vi "RT Driver VI.vi"(7 "Operation":T1, 11 "Device Reference in":T2 format="%.0x") -> (0 "Error Code":i32)   [LabVIEW 2020, in "AIM ARINC 429 Engine.lvlib" / "Custom Device.lvlib"]
uses:
  Custom Device.lvlib
  <vilib>/NI VeriStand/Custom Device API/Custom Device Item Ref.ctl
  <vilib>/NI VeriStand/Custom Device API/Hardware Interface Driver VI Operation.ctl
  Compiled.Settings.ctl
  Inline Execution Unit Compiled Information.ctl
  <vilib>/NI VeriStand/Custom Device API/Data Reference.ctl
  <vilib>/NI VeriStand/Custom Device API/Block Data Reference.ctl
  Asynchronous Execution Unit Compiled Information.ctl
  RTStateVariables.ctl
  <vilib>/NI/NIVS Inline Async API/_VS Inline Async API/VS Inline Async API/VS Inline Async API.lvclass
  Inline Execution Unit Runtime Information.ctl
  Interfaces/Execution Unit/Execution Unit.lvclass
  Asynchronous Execution Unit Runtime Information.ctl
  Interfaces/Shared Resources/Shared Resources.lvclass
  <vilib>/NI/NIVS Inline Async API/_VS Inline Async API/VS Inline Async API/VS Inline Async API.lvclass/VS Inline Async API.ctl
  <vilib>/NI/NIVS Inline Async API/_Data Access Engine/Data Access Engine/Data Access Engine.lvclass/Data Access Engine.ctl
  <vilib>/NI/NIVS Inline Async API/_Data Access Engine/Access Type Classes/Write/Write.lvclass/Write.ctl
  <vilib>/NI/NIVS Inline Async API/_Data Access Engine/Access Type Classes/ReadWrite/ReadWrite.lvclass/ReadWrite.ctl
  <vilib>/NI/NIVS Inline Async API/_Data Access Engine/Access Type Classes/Read/Read.lvclass/Read.ctl
  <vilib>/NI/NIVS Inline Async API/_Data Access Engine/Data Access Engine/Methods/Data.Engine.Read Data from HW.vi
  <vilib>/NI/NIVS Inline Async API/_VS Inline Async API/Error Handling Process/SubVIs/Error.GetError.vi
  <vilib>/NI/NIVS Inline Async API/_Data Access Engine/Data Access Engine/Methods/Data.Engine.Write Data to HW.vi
  <vilib>/NI/NIVS Inline Async API/_Data Access Engine/Access Type Classes/ReadWrite/ReadWrite.EngineData.vi
  <vilib>/NI/NIVS Inline Async API/_Data Access Engine/Access Type Classes/Write/Write.EngineData.vi
  <vilib>/NI/NIVS Inline Async API/_Data Access Engine/Access Type Classes/Read/Read.EngineData.vi
  <vilib>/NI VeriStand/Custom Device API/NI VeriStand - Get Channel Value by Data Reference.vi
  <vilib>/NI VeriStand/Custom Device API/NI VeriStand - Set Channel Value by Data Reference.vi
  <vilib>/NI VeriStand/Custom Device API/NI VeriStand - Get Channel Values by Block Data Reference.vi
  Scripting/AIM/Constants.vi
  <vilib>/NI VeriStand/Custom Device API/Get Item Property (Variant).vi
  <vilib>/NI VeriStand/Custom Device API/Global Data Refs.vi
  <vilib>/NI VeriStand/Custom Device API/Custom Device API.lvlib
  <vilib>/NI VeriStand/Custom Device Tools/Custom Device Utility Library/Custom Device Utility Library.lvlib
  Scripting/AIM/AIM ARINC 429 Scripting.lvlib
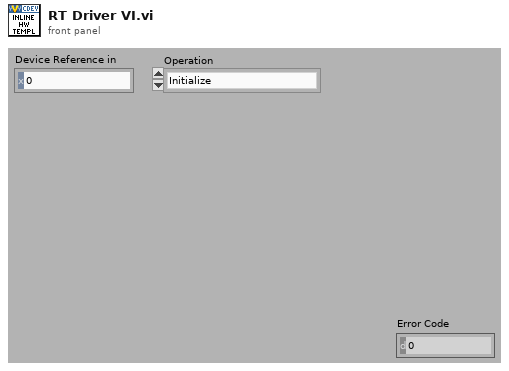
[diagram p1: front panel]
types:
  T1 = typedef "Custom Device API.lvlib/Hardware Interface Driver VI Operation.ctl" = enum16{"Initialize", "Start", "Read Data from HW", "Write Data to HW", "Close"}
  T2 = typedef "Custom Device API.lvlib/Custom Device Item Ref.ctl" = u64
  T3 = typedef "AIM ARINC 429 Engine.lvlib/Custom Device.lvlib/RTStateVariables.ctl" = cluster{"Async":refnum<class "VS Inline Async API.lvclass">, "Inline Execution Units":T4[], "Asynchronous Execution Units":cluster{"Grouped Asynchronous Execution Units":T7[]}[], "shared resources":refnum<class "Shared Resources.lvclass">}
  T4 = typedef "AIM ARINC 429 Engine.lvlib/Custom Device.lvlib/Inline Execution Unit Runtime Information.ctl" = cluster{"Execution Unit":refnum<class "Execution Unit.lvclass">, "Incoming Buffer":dbl[], "Outgoing Buffer":dbl[], "Incoming Data References":T5[], "Outgoing Data References":T6[]}
  T5 = typedef "Custom Device API.lvlib/Data Reference.ctl" = i32
  T6 = typedef "Custom Device API.lvlib/Block Data Reference.ctl" = cluster{"Data Reference":T5, "Offset":u64, "Length":u64}
  T7 = typedef "AIM ARINC 429 Engine.lvlib/Custom Device.lvlib/Asynchronous Execution Unit Runtime Information.ctl" = cluster{"Execution Unit":refnum<class "Execution Unit.lvclass">, "Incoming Channel Group Name":string, "Outgoing Channel Group Name":string, "ReadWrite Channel Group Name":string}
  T8 = typedef "AIM ARINC 429 Engine.lvlib/Custom Device.lvlib/Compiled.Settings.ctl" = cluster{"Name":string, "Inline Execution Unit Compiled Information":T9[], "Asynchronous Execution Unit Compiled Information":cluster{"Grouped Asynchronous Execution Unit Compiled Information":T10[]}[], "Flattened Shared Resources":string}
  T9 = typedef "AIM ARINC 429 Engine.lvlib/Custom Device.lvlib/Inline Execution Unit Compiled Information.ctl" = cluster{"Flattened Execution Unit":string, "Incoming Buffer":dbl[], "Outgoing Buffer":dbl[], "Incoming Data References":T5[], "Outgoing Data References":T6[]}
  T10 = typedef "AIM ARINC 429 Engine.lvlib/Custom Device.lvlib/Asynchronous Execution Unit Compiled Information.ctl" = cluster{"Flattened Execution Unit":string, "Incoming Channel Group Name":string, "Outgoing Channel Group Name":string, "ReadWrite Channel Group Name":string}
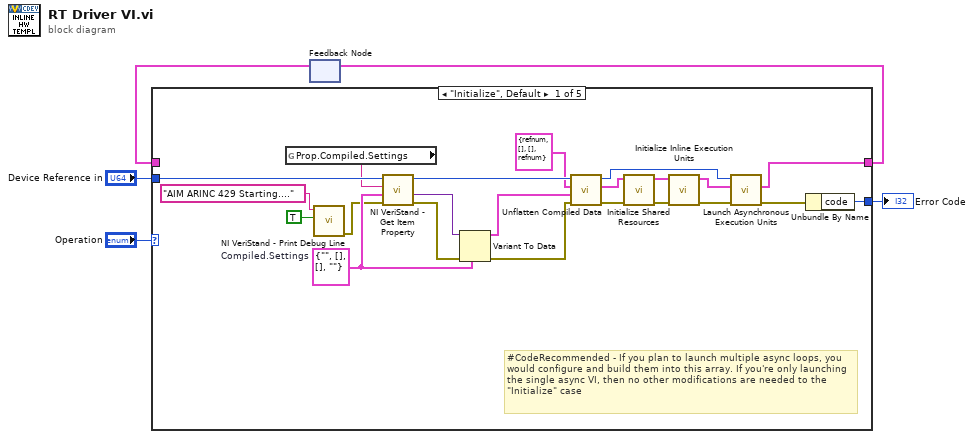
[diagram p0: block diagram]
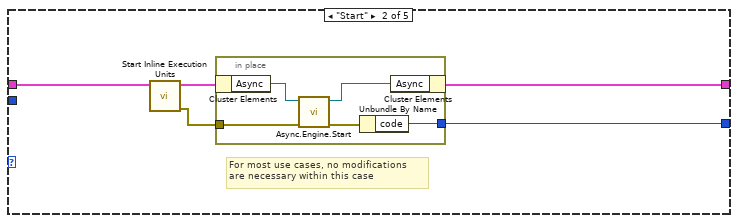
[diagram p2: hidden frame]
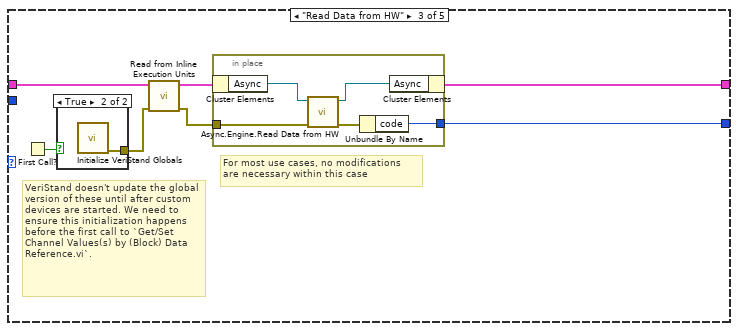
[diagram p3: hidden frame]
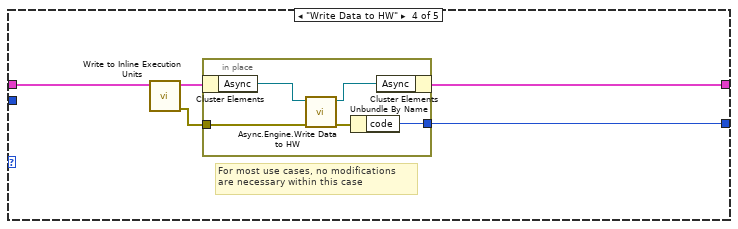
[diagram p5: hidden frame]
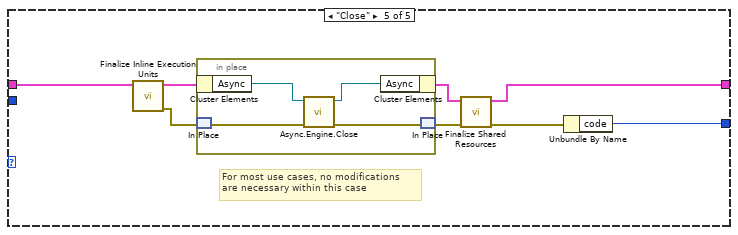
[diagram p6: hidden frame]
diagram:
  n1 = feedback #1() -> (w3:T3)  [unwired: 1 out]
  n2 = case shown="\"Initialize\", Default" "Operation" {
    tunnel: [w15 w31 w43 w54 w62] -> w4
    tunnel: w3 -> [_ w32 w42 w53 w68]
    tunnel: "Device Reference in" -> [w26 _ _ _ _]
    tunnel: [w27 w30 w44 w55 w65] -> w1
    frame "Initialize", Default {
      w22 = T8 {"Name"="", "Inline Execution Unit Compiled Information"=[], "Asynchronous Execution Unit Compiled Information"=[], "Flattened Shared Resources"=""}  # Compiled.Settings
      # "#CodeRecommended - If you plan to launch multiple async loops, you would configure and build them into this array. If you're only launching the single async VI, then no other modifications are needed to the \"Initialize\" case"
      n3 = global read "Constants.vi" "Prop.Compiled.Settings"() -> (w23:string)
      n4 = call <vilib>:"NI VeriStand - Print Debug Line.vi"("Add to log file? (F)"=TRUE, "Message"="AIM ARINC 429 Starting....") -> ("error out"=w21:errorcluster)  [unwired: 9 in]
      n5 = call-poly <vilib>:"NI VeriStand - Get Item Property.vi"("error in (no error)"=w21, "Default Value"=w22, "Property Name"=w23, "Item Ref in"=w26) -> ("error out"=w25:errorcluster, "Value"=w24:variant, "Item Ref out"=w17:T2)  [unwired: 4 in, 1 out]
      n6 = Variant To Data(error in=w25, type=w22, Variant=w24) -> (data=w19:T8, error out=w18:errorcluster)
      n7 = call "Unflatten Compiled Data.vi"("error in (no error)"=w18, "Compiled.Settings"=w19, "RTStateVariables in"=T3 {"Async"=refnum, "Inline Execution Units"=[], "Asynchronous Execution Units"=[], "shared resources"=refnum} ("RTStateVariables"), "Item Ref in"=w17) -> ("error out"=w9:errorcluster, "RTStateVariables out"=w11:T3, "Item Ref out"=w14:T2)  [unwired: 5 in]
      n8 = call "Initialize Shared Resources.vi"("error in"=w9, "RTStateVariables in"=w11) -> ("error out"=w8:errorcluster, "RTStateVariables out"=w12:T3)  [unwired: 8 in]
      n9 = call "Initialize Inline Execution Units.vi"("error in"=w8, "RTStateVariables in"=w12) -> ("error out"=w7:errorcluster, "RTStateVariables out"=w13:T3)  [unwired: 8 in]
      n10 = call "Launch Asynchronous Execution Units.vi"("error in (no error)"=w7, "RTStateVariables in"=w13, "Device Ref in"=w14) -> ("error out"=w6:errorcluster, "RTStateVariables out"=w15:T3)  [unwired: 6 in, 1 out]
      n11 = Unbundle By Name(w6) -> ("code"=w27:i32)
    }
    frame "Start" {
      # "For most use cases, no modifications \nare necessary within this case"
      n12 = call "Start Inline Execution Units.vi"("RTStateVariables in"=w32) -> ("error out"=w28:errorcluster, "RTStateVariables out"=w29:T3)  [unwired: 9 in]
      n13 = in-place {
        in-place-border: [w34] -> w30
        in-place-border: w28 -> [w33]
        n14 = in-place-cluster #2(w29) -> ("Async"=w37:refnum<class "VS Inline Async API.lvclass">)
        n15 = call <vilib>:"Async.Engine.Start.vi"("error in (no error)"=w33, "VS Inline Async API in"=w37) -> ("error out"=w35:errorcluster, "VS Inline Async API out"=w36:refnum<class "VS Inline Async API.lvclass">)  [unwired: 8 in]
        n16 = Unbundle By Name(w35) -> ("code"=w34:i32)
        n17 = in-place-cluster #2("Async"=w36) -> (w31:T3)
      }
    }
    frame "Read Data from HW" {
      # "VeriStand doesn't update the global version of these until after custom devices are started. We need to ensure this initialization happens before the first call to `Get/Set Channel Values(s) by (Block) Data Reference.vi`."
      # "For most use cases, no modifications \nare necessary within this case"
      n18 = First Call?() -> (First Call?: T/F=w39:bool)
      n19 = case shown="True" w39 {
        tunnel: [_ w45] -> w38
        frame False {
        }
        frame True {
          n20 = call "Initialize VeriStand Globals.vi"() -> ("error out"=w45:errorcluster)  [unwired: 11 in]
        }
      }
      n21 = call "Read from Inline Execution Units.vi"("error in (no error)"=w38, "RTStateVariables in"=w42) -> ("error out"=w40:errorcluster, "RTStateVariables out"=w41:T3)  [unwired: 8 in]
      n22 = in-place {
        in-place-border: [w48] -> w44
        in-place-border: w40 -> [w46]
        n23 = in-place-cluster #3(w41) -> ("Async"=w50:refnum<class "VS Inline Async API.lvclass">)
        n24 = call <vilib>:"Async.Engine.Read Data from HW.vi"("error in"=w46, "Async in"=w50) -> ("error out"=w47:errorcluster, "Async out"=w49:refnum<class "VS Inline Async API.lvclass">)  [unwired: 8 in]
        n25 = Unbundle By Name(w47) -> ("code"=w48:i32)
        n26 = in-place-cluster #3("Async"=w49) -> (w43:T3)
      }
    }
    frame "Write Data to HW" {
      # "For most use cases, no modifications \nare necessary within this case"
      n27 = call "Write to Inline Execution Units.vi"("RTStateVariables in"=w53) -> ("error out"=w51:errorcluster, "RTStateVariables out"=w52:T3)  [unwired: 9 in]
      n28 = in-place {
        in-place-border: [w60] -> w55
        in-place-border: w51 -> [w56]
        n29 = in-place-cluster #4(w52) -> ("Async"=w58:refnum<class "VS Inline Async API.lvclass">)
        n30 = call <vilib>:"Async.Engine.Write Data to HW.vi"("error in (no error)"=w56, "VS Inline Async API in"=w58) -> ("error out"=w59:errorcluster, "VS Inline Async API out"=w57:refnum<class "VS Inline Async API.lvclass">)  [unwired: 8 in]
        n31 = Unbundle By Name(w59) -> ("code"=w60:i32)
        n32 = in-place-cluster #4("Async"=w57) -> (w54:T3)
      }
    }
    frame "Close" {
      # "For most use cases, no modifications \nare necessary within this case"
      n33 = call "Finalize Inline Execution Units.vi"("RTStateVariables in"=w68) -> ("error out"=w66:errorcluster, "RTStateVariables out"=w67:T3)  [unwired: 9 in]
      n34 = in-place {
        n35 = in-place-cluster #5(w67) -> ("Async"=w72:refnum<class "VS Inline Async API.lvclass">)
        n36 = in-place-match #6(w66) -> (w70:errorcluster)
        n37 = call <vilib>:"Async.Engine.Close.vi"("error in (no error)"=w70, "Async in"=w72) -> ("error out"=w69:errorcluster, "Async out"=w71:refnum<class "VS Inline Async API.lvclass">)  [unwired: 8 in]
        n38 = in-place-cluster #5("Async"=w71) -> (w63:T3)
        n39 = in-place-match #6(w69) -> (w64:errorcluster)
      }
      n40 = call "Finalize Shared Resources.vi"("error in"=w64, "RTStateVariables in"=w63) -> ("error out"=w61:errorcluster, "RTStateVariables out"=w62:T3)  [unwired: 8 in]
      n41 = Unbundle By Name(w61) -> ("code"=w65:i32)
    }
  }
  "Error Code" <- w1
  n42 = feedback-in #1(w4) -> ()
